vi "FuncVI_Sub - VI - Get VI control value.vi"(5 "expected type":T1=enum."DBL Number", 6 "error in":errorcluster, 8 "control name":string, 9 "VI Ref":refnum<vi>) -> (0 "error out":errorcluster, 2 "str":string, 3 "dup VI Ref":refnum<vi>, 4 "type":T1=enum."DBL Number")   [LabVIEW 2021]
doc: "::: CalcExpress Toolkit :::\nCopyright (c) 2000-2026 Konstantin Shifershteyn. All rights reserved."
uses:
  cetypes.llb/CalcExpress Data Type.ctl
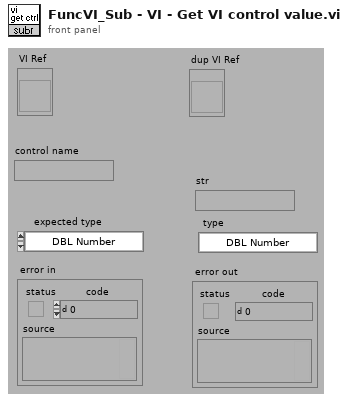
[diagram p1: front panel]
types:
  T1 = typedef "CalcExpress Data Type.ctl" = enum32{"String", "DBL Number", "identifier", "1D Array of DBL", "2D Array of DBL", "CDB Number", "1D Array of CDB", "2D Array of CDB", "1D Array of String", "2D Array of String", "Unknown data type"}
  T2 = enum32{"String", "DBL Number", "identifier", "1D Array of DBL", "2D Array of DBL", "CDB Number", "1D Array of CDB", "2D Array of CDB", "1D Array of String", "2D Array of String", "Unknown data type"}
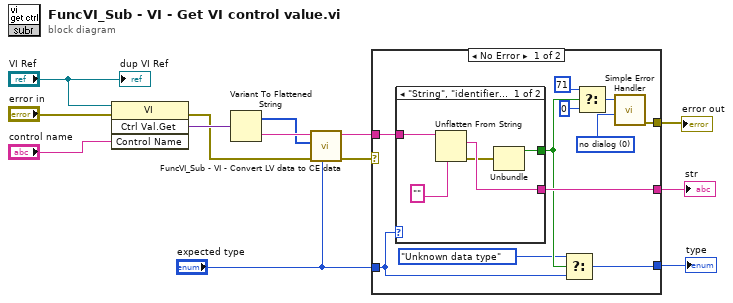
[diagram p0: block diagram]
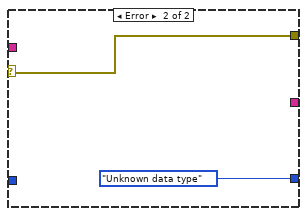
[diagram p3: hidden frame]
diagram:
  n1 = invoke class="VI" method="Ctrl Val.Get"(reference="VI Ref", error in="error in", "Control Name"="control name") -> (error out=w4:errorcluster, "Get Control Value Variant"=w8:variant)  [unwired: 1 in, 2 out]
  n2 = Variant To Flattened String(Variant=w8) -> (data string=w6:string, 1:w5:i16[])
  n3 = call "FuncVI_Sub - VI - Convert LV data to CE data.vi"("CE data type"="expected type", "error in"=w4, "LV Type Descriptor"=w5, "flattened data in"=w6) -> ("error out"=w7:errorcluster, "flattened data out"=w9:string)  [unwired: 4 in]
  n4 = case shown="No Error" w7 {
    selector: w7 -> [_ w31]
    tunnel: "expected type" -> [w16 _]
    tunnel: w9 -> [w24 _]
    tunnel: [w23 _] -> w13
    tunnel: [w18 T2."Unknown data type" ("expected type")] -> w12
    tunnel: [w20 w31] -> w11
    frame No Error {
      w14 = 0 items=["no dialog", "OK message", "continue or stop message"] ("type of dialog (OK msg:1)")
      n5 = case shown="\"String\", \"identifier\"" w16 {
        tunnel: w24 -> [w29 w30]
        tunnel: [w28 w30] -> w23
        tunnel: [w26 _] -> w17
        frame "String", "identifier" {
          n6 = Unflatten From String(type="", binary string=w29) -> (value=w28:string, error out=w25:errorcluster)  [unwired: 3 in, 1 out]
          n7 = Unbundle(w25) -> ("status"=w26:bool)  [unwired: 2 out]
        }
        frame "DBL Number", Default {
        }
      }
      n8 = Select(t=T2."Unknown data type", s=w17, f=w16) -> (s? t:f=w18:T1)
      n9 = Select(t=71, s=w17, f=0) -> (s? t:f=w19:i32)
      n10 = call <vilib>:"Simple Error Handler.vi"("error code (no error:0)"=w19, "type of dialog (OK msg:1)"=w14) -> ("error out"=w20:errorcluster)  [unwired: 3 in, 4 out]
    }
    frame Error {
    }
  }
  "str" <- w13
  "error out" <- w11
  "type" <- w12
  "dup VI Ref" <- "VI Ref"
